vi "Test - Format Entries.vi"(8 "error in":errorcluster, 10 "Original ID":string, 11 "Entries":T1) -> (0 "error out":errorcluster, 3 "Text":string)   [LabVIEW 2026]
doc: "Test support. Formats time entries as one comparable text, one line per entry, each line ending in a semicolon: tag|Project ID|Task ID|Start|End|Description. Start and End are seconds since 1904 (UTC) with 3 decimals and a period as the decimal point; a running entry's End is 0.000. The tag replaces the random ID: orig when the ID is Original ID, none when it is empty, new otherwise.\n\nInputs: Entries; Original ID; error in (passed through). Outputs: Text; error out.\n\nGenerated by: Claude"
uses:
  Storage/Rows/Time Entry.ctl
  Storage/Rows/Time Entry List.ctl
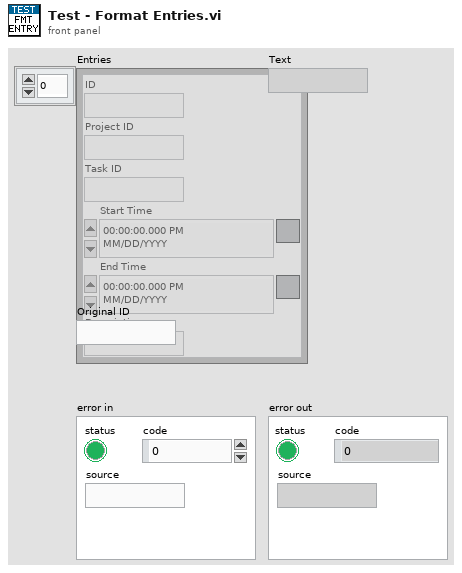
[diagram p1: front panel]
types:
  T1 = typedef "Time Entry List.ctl" = T2[]
  T2 = typedef "Time Entry.ctl" = cluster{"ID":string, "Project ID":string, "Task ID":string, "Start Time":timestamp, "End Time":timestamp, "Description":string}
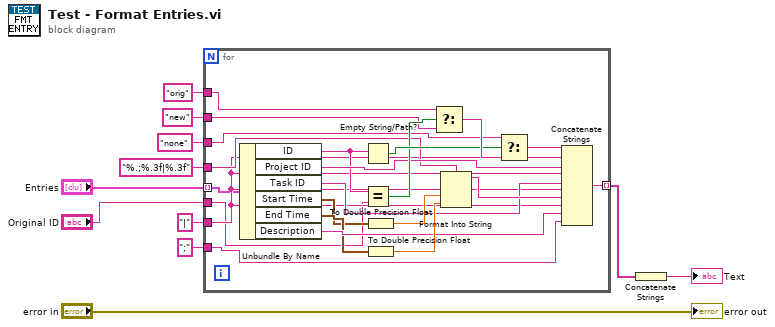
[diagram p0: block diagram]
diagram:
  n1 = for {
    tunnel: "Entries" -> [w12] mode=indexing
    tunnel: "Original ID" -> [w13]
    tunnel: "|" ("bar") -> [w14]
    tunnel: ";" ("semicolon") -> [w15]
    tunnel: "%.;%.3f|%.3f" ("times format") -> [w16]
    tunnel: "orig" ("orig") -> [w17]
    tunnel: "new" ("new") -> [w18]
    tunnel: "none" ("none") -> [w19]
    tunnel: [w33] -> w11 mode=indexing
    n2 = Unbundle By Name(w12) -> ("ID"=w20:string, "Project ID"=w21:string, "Task ID"=w22:string, "Start Time"=w23:timestamp, "End Time"=w24:timestamp, "Description"=w25:string)
    n3 = Empty String/Path?(string/path=w20) -> (empty?=w27:bool)
    n4 = Equal?(x=w20, y=w13) -> (x = y?=w26:bool)
    n5 = To Double Precision Float(number=w23) -> (double precision float=w30:dbl)
    n6 = To Double Precision Float(number=w24) -> (double precision float=w31:dbl)
    n7 = Select(t=w17, s=w26, f=w18) -> (s? t:f=w28:string)
    n8 = Format Into String(format string=w16, w30, w31) -> (resulting string=w32:string)  [unwired: 2 in, 1 out]
    n9 = Select(t=w19, s=w27, f=w28) -> (s? t:f=w29:string)
    n10 = Concatenate Strings(w29, w14, w21, w14, w22, w14, w32, w14, w25, w15) -> (w33:string)
  }
  n11 = Concatenate Strings(w11) -> (→"Text":string)
  "error out" <- "error in"
